vi "Low-Level Read.vi"(8 "error in (no error)":errorcluster, 9 "timeout ms (5000)":i32=5000, 11 "WebSockets in":refnum<class "WebSocket.lvclass">) -> (0 "error out":errorcluster, 1 "Opcode":T1=1 items=["Cont. Frame"=0, "Text"=1, "Binary"=2, "Ping"=9, "Pong"=10], 2 "Data":u8[](array[numeric]), 3 "WebSockets out":refnum<class "WebSocket.lvclass">, 4 "Finished?":bool)   [LabVIEW 2013, in "WebSockets.lvlib" / "WebSocket.lvclass"]
doc: "Reads and decodes an incoming WebSockets frame.\n\nOpcode: Opcode for the message.\nData: Contains the WebSockets payload\nFinished?: Determines whether the message is complete for fragmented messages. If false, must continue to read messages (continuation frames with opcode = 0) until Finished? is true."
uses:
  WebSocket.lvclass
  Opcodes.ctl
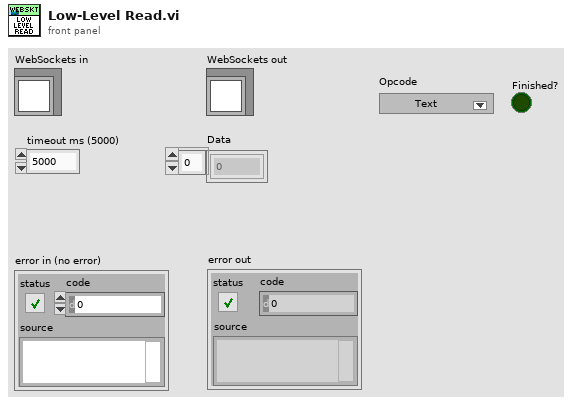
[diagram p1: front panel]
types:
  T1 = typedef "WebSockets.lvlib/WebSocket.lvclass/Opcodes.ctl" = u8
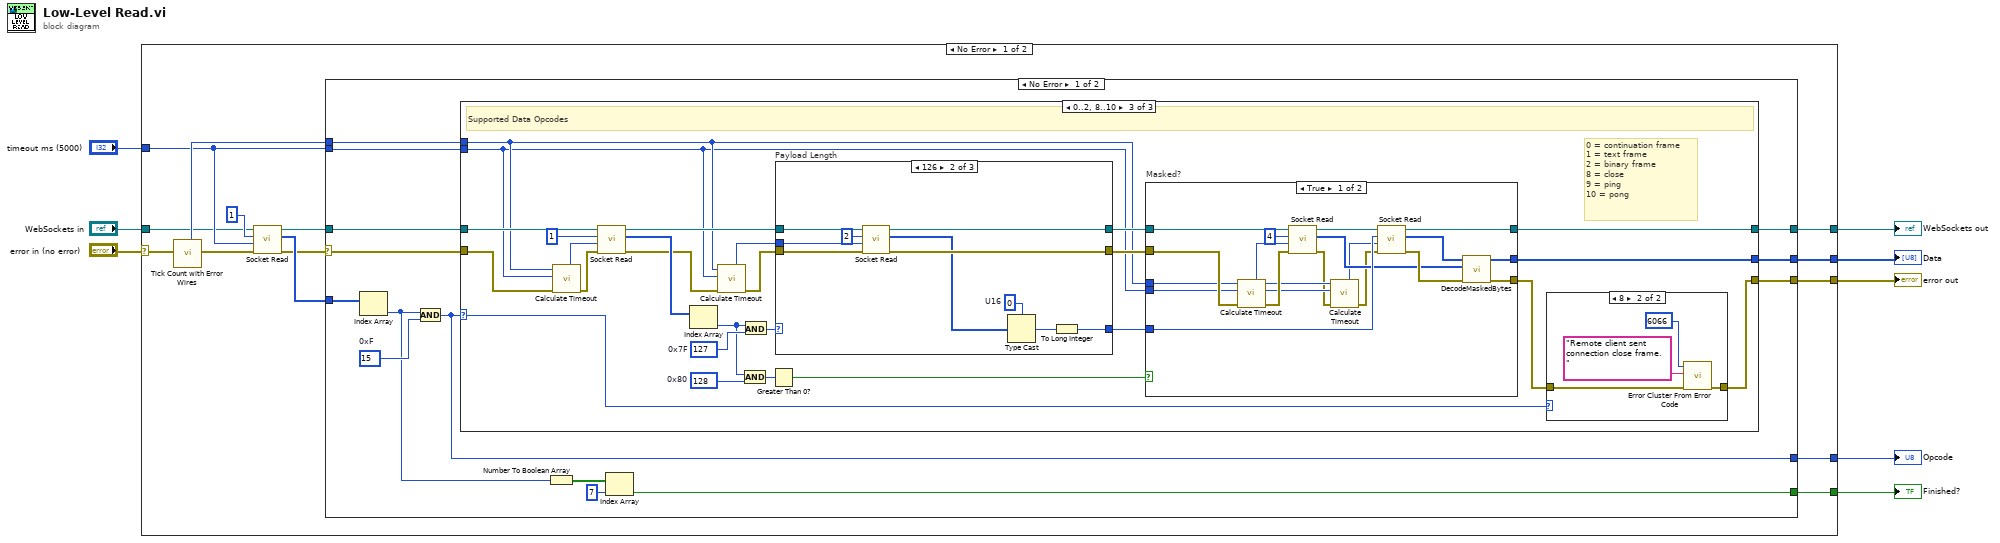
[diagram p0: block diagram]
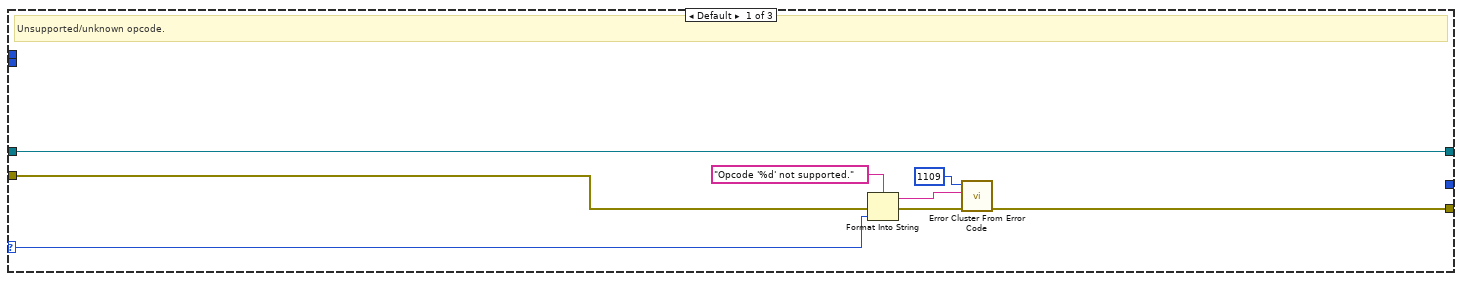
[diagram p2: hidden frame]
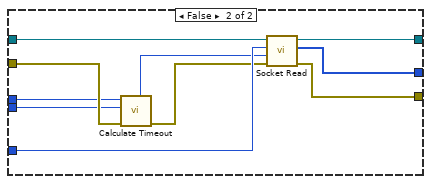
[diagram p5: hidden frame]
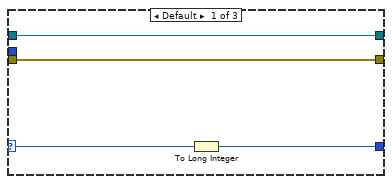
[diagram p6: hidden frame]
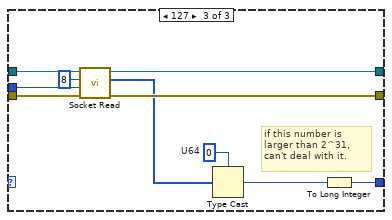
[diagram p7: hidden frame]
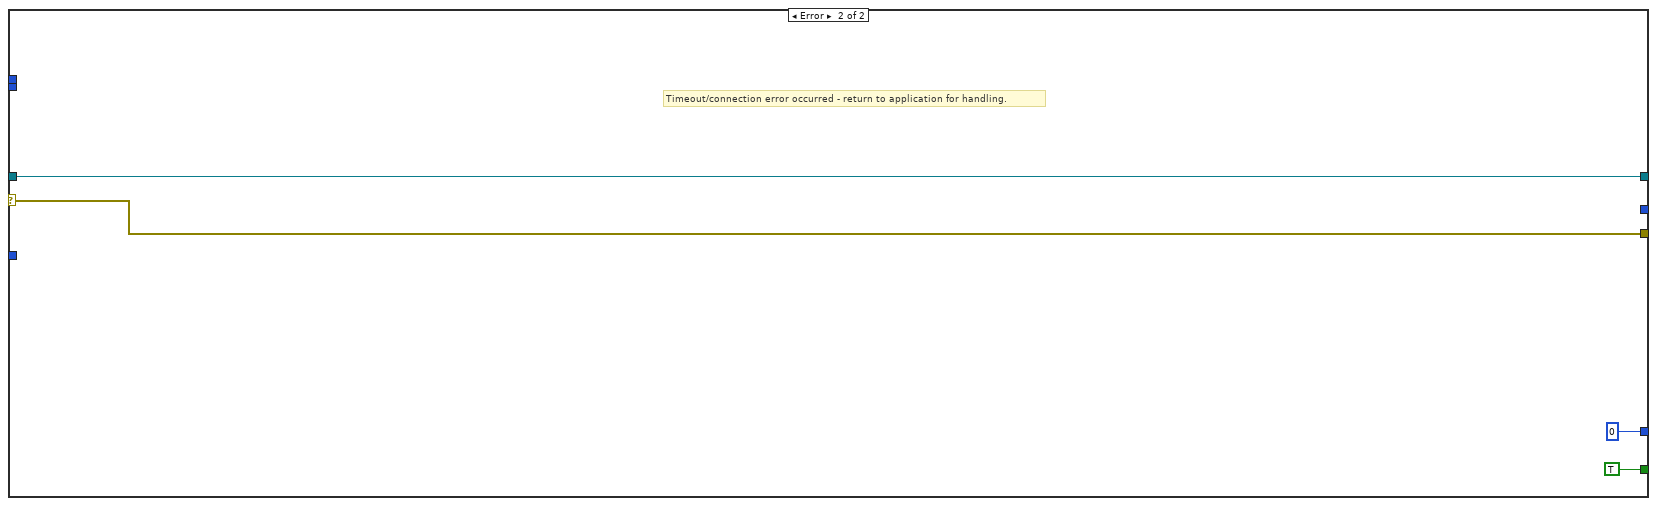
[diagram p8: hidden frame]
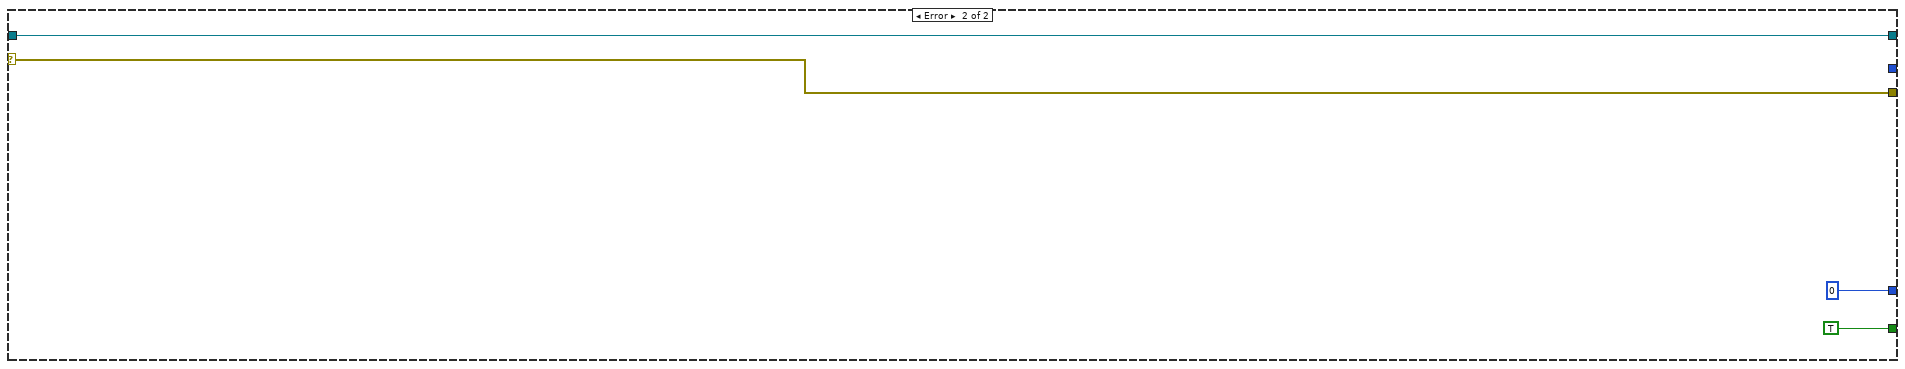
[diagram p9: hidden frame]
diagram:
  n1 = case shown="No Error" "error in (no error)" {
    selector: "error in (no error)" -> [w18 w137]
    tunnel: [w22 _] -> w3
    tunnel: [w21 w137] -> w7
    tunnel: "timeout ms (5000)" -> [w14 _]
    tunnel: [w20 u8 0] -> w4
    tunnel: [w19 TRUE] -> w5
    tunnel: "WebSockets in" -> [w10 w134]
    tunnel: [w9 w134] -> w1
    frame No Error {
      n2 = call "Tick Count with Error Wires.vi"("error in (no error)"=w18) -> ("error out"=w16:errorcluster, "millisecond timer value"=w17:u32)  [unwired: 9 in]
      n3 = call "Socket Read.vi"("error in (no error)"=w16, "timeout ms (5000)"=w14, "# bytes to read"=1 ("bytes to read"), "WebSocket in"=w10) -> ("error out"=w12:errorcluster, "Read Bytes"=w13:u8[], "WebSocket out"=w11:refnum<class "WebSocket.lvclass">)  [unwired: 5 in]
      n4 = case shown="No Error" w12 {
        selector: w12 -> [w32 w132]
        tunnel: w13 -> [w24 _]
        tunnel: w11 -> [w36 w133]
        tunnel: [w35 w133] -> w9
        tunnel: [w34 _] -> w22
        tunnel: [w33 w132] -> w21
        tunnel: [w30 u8 0] -> w20
        tunnel: [w27 TRUE] -> w19
        tunnel: w14 -> [w26 _]
        tunnel: w17 -> [w23 _]
        frame No Error {
          w31 = u8 15  # 0xF
          n5 = Index Array(array=w24) -> (element=w29:u8)  [unwired: 1 in]
          n6 = And(x=w29, y=w31) -> (x .and. y?=w30:u8)
          n7 = case shown="0..2, 8..10" w30 {
            selector: w30 -> [w38 _ w59]
            tunnel: w36 -> [w44 w45 w65]
            tunnel: [w44 w45 w72] -> w35
            tunnel: [_ _ w66] -> w34
            tunnel: [w43 w46 w57] -> w33
            tunnel: w32 -> [w42 w46 w54]
            tunnel: w26 -> [_ _ w47]
            tunnel: w23 -> [_ _ w48]
            frame Default {
              # "Unsupported/unknown opcode."
              n8 = Format Into String(format string="Opcode '%d' not supported.", error in=w42, w38) -> (resulting string=w40:string, error out=w41:errorcluster)  [unwired: 1 in]
              n9 = call <vilib>:"Error Cluster From Error Code.vi"("error in (no error)"=w41, "error message (\"\")"=w40, "error code (0)"=1109) -> ("error out"=w43:errorcluster)  [unwired: 6 in]
            }
            frame 3..7, 11..15 {
              # "3-7: Reserved non-control frames\n11-15: Reserved control frames"
              # "Reserved opcodes"
            }
            frame 0..2, 8..10 {
              w62 = u8 128  # 0x80
              w71 = u8 127  # 0x7F
              # "0 = continuation frame\n1 = text frame\n2 = binary frame\n8 = close\n9 = ping\n10 = pong"
              # "Supported Data Opcodes"
              n10 = call "Calculate Timeout.vi"("error in (no error)"=w54, "timeout ms"=w47, "t0"=w48) -> ("error out"=w53:errorcluster, "new timeout ms"=w51:i32)  [unwired: 6 in, 1 out]
              n11 = call "Socket Read.vi"("error in (no error)"=w53, "timeout ms (5000)"=w51, "# bytes to read"=1 ("bytes to read"), "WebSocket in"=w65) -> ("error out"=w52:errorcluster, "Read Bytes"=w56:u8[], "WebSocket out"=w64:refnum<class "WebSocket.lvclass">)  [unwired: 5 in]
              n12 = Index Array(array=w56) -> (element=w55:u8)  [unwired: 1 in]
              n13 = call "Calculate Timeout.vi"("error in (no error)"=w52, "timeout ms"=w47, "t0"=w48) -> ("error out"=w50:errorcluster, "new timeout ms"=w49:i32)  [unwired: 6 in, 1 out]
              n14 = And(x=w55, y=w62) -> (x .and. y?=w61:u8)
              n15 = And(x=w55, y=w71) -> (x .and. y?=w70:u8)
              n16 = Greater Than 0?(x=w61) -> (x > 0?=w60:bool)
              n17 = case "Payload Length" shown="126" w70 {
                selector: w70 -> [w108 _ _]
                tunnel: w64 -> [w109 w119 w128]
                tunnel: [w109 w118 w127] -> w69
                tunnel: [w107 w113 w126] -> w67
                tunnel: [w106 w116 w125] -> w68
                tunnel: w50 -> [w106 w115 w124]
                tunnel: w49 -> [_ w110 w120]
                frame Default {
                  n18 = To Long Integer(number=w108) -> (32bit integer=w107:i32)
                }
                frame 126 {
                  w112 = u16 0  # U16
                  n19 = call "Socket Read.vi"("error in (no error)"=w115, "timeout ms (5000)"=w110, "# bytes to read"=2 ("bytes to read"), "WebSocket in"=w119) -> ("error out"=w116:errorcluster, "Read Bytes"=w114:u8[], "WebSocket out"=w118:refnum<class "WebSocket.lvclass">)  [unwired: 5 in]
                  n20 = Type Cast(type=w112, x=w114) -> (*(type *) &x=w111:u16)
                  n21 = To Long Integer(number=w111) -> (32bit integer=w113:i32)
                }
                frame 127 {
                  w123 = u64 0  # U64
                  # "if this number is larger than 2^31, can't deal with it."
                  n22 = call "Socket Read.vi"("error in (no error)"=w124, "timeout ms (5000)"=w120, "# bytes to read"=8 ("bytes to read"), "WebSocket in"=w128) -> ("error out"=w125:errorcluster, "Read Bytes"=w121:u8[], "WebSocket out"=w127:refnum<class "WebSocket.lvclass">)  [unwired: 5 in]
                  n23 = Type Cast(type=w123, x=w121) -> (*(type *) &x=w122:u64)
                  n24 = To Long Integer(number=w122) -> (32bit integer=w126:i32)
                }
              }
              n25 = case "Masked?" shown="True" w60 {
                tunnel: [w95 w105] -> w72
                tunnel: w69 -> [w94 w104]
                tunnel: w68 -> [w85 w100]
                tunnel: w67 -> [w91 w103]
                tunnel: [w89 w101] -> w66
                tunnel: [w87 w102] -> w58
                tunnel: w48 -> [w82 w97]
                tunnel: w47 -> [w81 w96]
                frame True {
                  n26 = call "Calculate Timeout.vi"("error in (no error)"=w85, "timeout ms"=w81, "t0"=w82) -> ("error out"=w84:errorcluster, "new timeout ms"=w83:i32)  [unwired: 6 in, 1 out]
                  n27 = call "Socket Read.vi"("error in (no error)"=w84, "timeout ms (5000)"=w83, "# bytes to read"=4 ("bytes to read"), "WebSocket in"=w94) -> ("error out"=w80:errorcluster, "Read Bytes"=w86:u8[], "WebSocket out"=w93:refnum<class "WebSocket.lvclass">)  [unwired: 5 in]
                  n28 = call "Calculate Timeout.vi"("error in (no error)"=w80, "timeout ms"=w81, "t0"=w82) -> ("error out"=w79:errorcluster, "new timeout ms"=w78:i32)  [unwired: 6 in, 1 out]
                  n29 = call "Socket Read.vi"("error in (no error)"=w79, "timeout ms (5000)"=w78, "# bytes to read"=w91, "WebSocket in"=w93) -> ("error out"=w88:errorcluster, "Read Bytes"=w90:u8[], "WebSocket out"=w95:refnum<class "WebSocket.lvclass">)  [unwired: 5 in]
                  n30 = call "DecodeMaskedBytes.vi"("error in (no error)"=w88, "Mask Bytes"=w86, "Encoded Data"=w90) -> ("error out"=w87:errorcluster, "Decoded Data"=w89:u8[])  [unwired: 7 in]
                }
                frame False {
                  n31 = call "Calculate Timeout.vi"("error in (no error)"=w100, "timeout ms"=w96, "t0"=w97) -> ("error out"=w98:errorcluster, "new timeout ms"=w99:i32)  [unwired: 6 in, 1 out]
                  n32 = call "Socket Read.vi"("error in (no error)"=w98, "timeout ms (5000)"=w99, "# bytes to read"=w103, "WebSocket in"=w104) -> ("error out"=w102:errorcluster, "Read Bytes"=w101:u8[], "WebSocket out"=w105:refnum<class "WebSocket.lvclass">)  [unwired: 5 in]
                }
              }
              n33 = case shown="8" w59 {
                tunnel: w58 -> [w73 w75]
                tunnel: [w73 w74] -> w57
                frame Default {
                }
                frame 8 {
                  n34 = call <vilib>:"Error Cluster From Error Code.vi"("error in (no error)"=w75, "error message (\"\")"="Remote client sent connection close frame." ("error message (\"\")"), "error code (0)"=6066) -> ("error out"=w74:errorcluster)  [unwired: 6 in]
                }
              }
            }
          }
          n35 = Number To Boolean Array(number=w29) -> (Boolean array=w28:bool[])
          n36 = Index Array(array=w28, index=7) -> (element=w27:bool)
        }
        frame Error {
          # "Timeout/connection error occurred - return to application for handling."
        }
      }
    }
    frame Error {
    }
  }
  "error out" <- w7
  "Finished?" <- w5
  "Opcode" <- w4
  "Data" <- w3
  "WebSockets out" <- w1
